vi "Calc Velocity Setpoints.vi"(7 "Autos":T6, 8 "Iterations":i32, 9 "Angle":dbl, 10 "V Scale":dbl=1.0) -> (0 "tick count(ms)":u32, 1 "Finished?":bool, 2 "setpoints":cluster{"left":dbl, "right":dbl})   [LabVIEW 2023]
uses:
  bordeaux-main/Bordeaux/Types/Single Cmd Info.ctl
  <vilib>/picture/picture.llb/imagedata.ctl
  bordeaux-main/Bordeaux/Types/Trajectory Data.ctl
  bordeaux-main/Bordeaux/Types/Segment Type.ctl
  <vilib>/addons/control/pid/pid.llb/PID (DBL).vi
  <vilib>/addons/control/pid/NI_PID_pid.lvlib
panel:
  in  "IMU PID":T1={"proportional gain (Kc)"=0.06, "integral time (Ti, min)"=0.0, "derivative time (Td, min)"=0.001}
  in  "Turn Scale":dbl=1.0
  in  "Half Track Width (ft)":dbl=0.9
  in  "IMU Correction":bool=TRUE
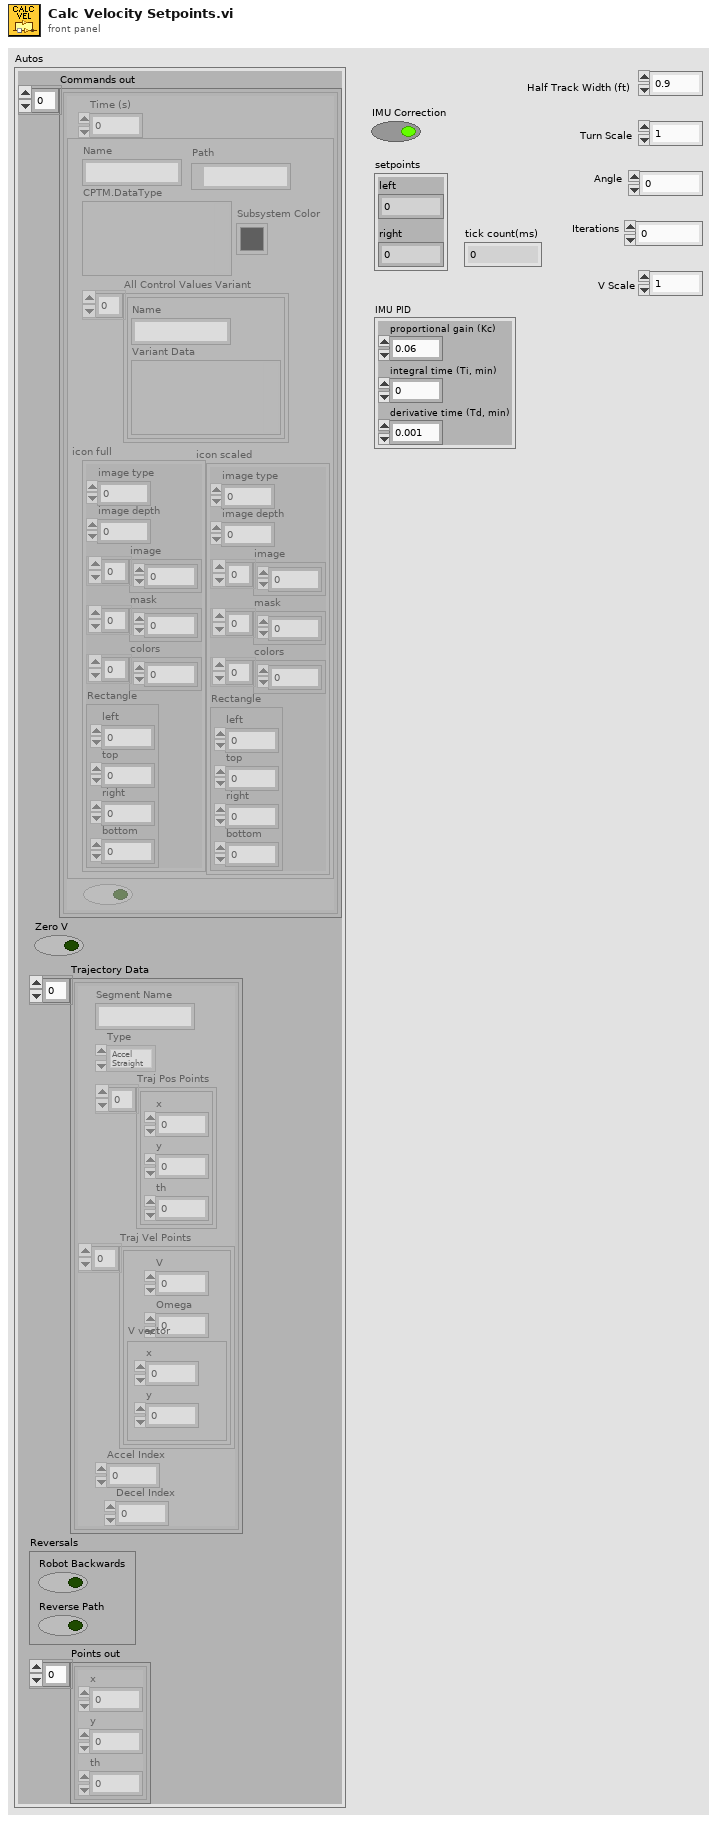
[diagram p1: front panel]
types:
  T1 = cluster{"proportional gain (Kc)":dbl, "integral time (Ti, min)":dbl, "derivative time (Td, min)":dbl}
  T2 = typedef "Single Cmd Info.ctl" = cluster{"Name":string, "CPTM.DataType":variant, "All Control Values Variant":cluster{"Name":string, "Variant Data":variant}[], "icon full":T3, "icon scaled":T3, "Path":path, "Subsystem Color":u32}
  T3 = typedef "imagedata.ctl" = cluster{"image type":i32, "image depth":i32, "image":u8[], "mask":u8[], "colors":u32[], "Rectangle":cluster{"left":i16, "top":i16, "right":i16, "bottom":i16}}
  T4 = typedef "Trajectory Data.ctl" = cluster{"Segment Name":string, "Type":T5, "Traj Pos Points":cluster{"x":dbl, "y":dbl, "th":dbl}[], "Traj Vel Points":cluster{"V":dbl, "Omega":dbl, "V vector":cluster{"y":dbl, "x":dbl}}[], "Accel Index":i32, "Decel Index":i32}[]
  T5 = typedef "Segment Type.ctl" = enum16{"Accel Straight", "Const Straight", "Blend", "Circle", "Bezier"}
  T6 = cluster{"Commands out":cluster{"Time (s)":dbl, T2, bool}[], "Zero V":bool, "Trajectory Data":T4, "Reversals":cluster{"Robot Backwards":bool, "Reverse Path":bool}, "Points out":cluster{"x":dbl, "y":dbl, "th":dbl}[]}
  T7 = cluster{"Robot Backwards":bool, "Reverse Path":bool}
  T8 = cluster{"V":dbl, "Omega":dbl, "V vector":cluster{"y":dbl, "x":dbl}}[]
  T9 = cluster{"V":dbl, "Omega":dbl, "V vector":cluster{"y":dbl, "x":dbl}}
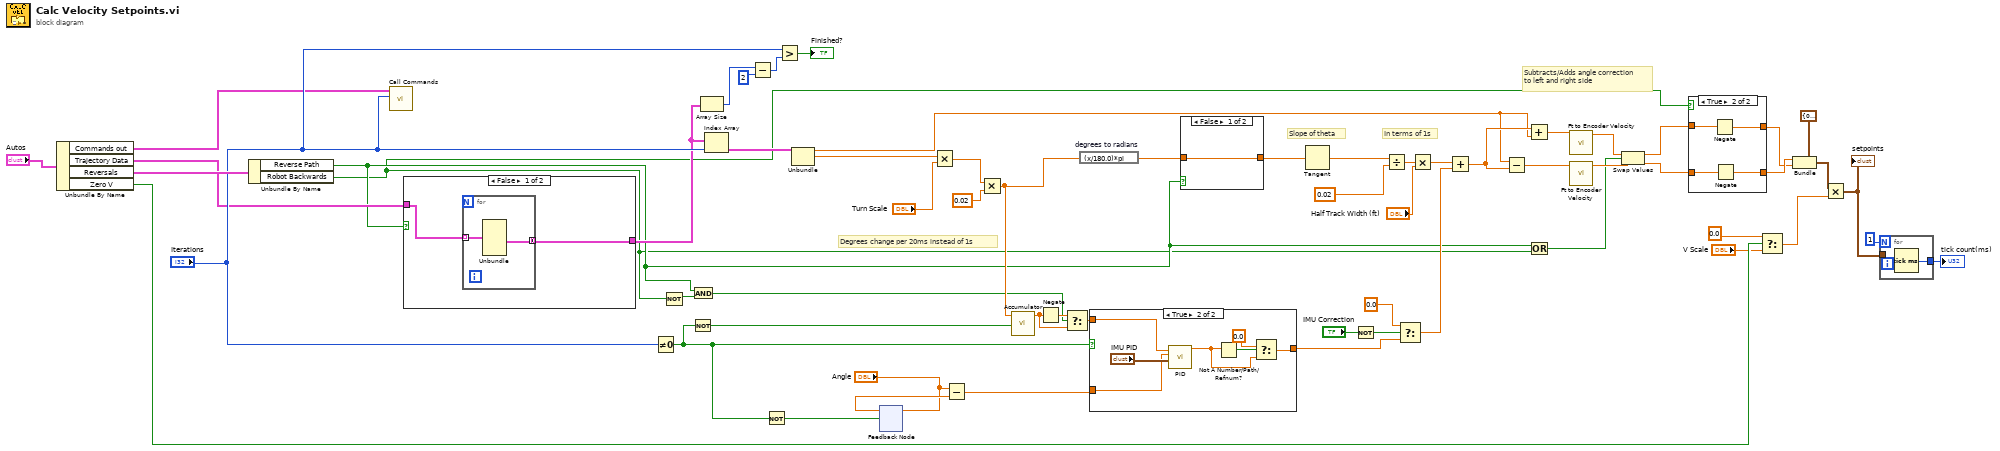
[diagram p0: block diagram]
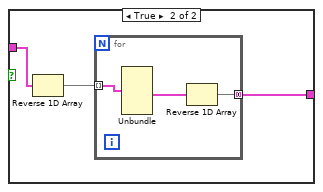
[diagram p2: hidden frame]
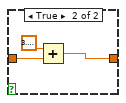
[diagram p3: hidden frame]
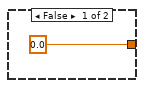
[diagram p4: hidden frame]
diagram:
  # "In terms of 1s"
  # "Slope of theta"
  # "Subtracts/Adds angle correction\nto left and right side"
  # "Degrees change per 20ms instead of 1s"
  n1 = Unbundle By Name("Autos") -> ("Commands out"=w18:cluster{"Time (s)":dbl, T2, bool}[], "Trajectory Data"=w30:T4, "Reversals"=w40:T7, "Zero V"=w17:bool)
  n2 = Unbundle By Name(w40) -> ("Reverse Path"=w3:bool, "Robot Backwards"=w2:bool)
  n3 = call "Call Commands.vi"("Iterations"="Iterations", "Commands"=w18) -> ()  [unwired: 10 in]
  n4 = case shown="False" w3 {
    tunnel: w30 -> [w63 w68]
    tunnel: [w62 w66] -> w32
    frame False {
      n5 = for {
        tunnel: w63 -> [w65] mode=indexing
        tunnel: [w64] -> w62 mode=concatenating
        n6 = Unbundle(w65) -> ("Traj Vel Points"=w64:T8)  [unwired: 5 out]
      }
    }
    frame True {
      n7 = Reverse 1D Array(array=w68) -> (reversed array=w67:T4)
      n8 = for {
        tunnel: w67 -> [w71] mode=indexing
        tunnel: [w69] -> w66 mode=concatenating
        n9 = Unbundle(w71) -> ("Traj Vel Points"=w70:T8)  [unwired: 5 out]
        n10 = Reverse 1D Array(array=w70) -> (reversed array=w69:T8)
      }
    }
  }
  n11 = Not Equal To 0?(x="Iterations") -> (x != 0?=w48:bool)
  n12 = Not(x=w2) -> (.not. x?=w8:bool)
  n13 = Not(x=w48) -> (.not. x?=w47:bool)
  n14 = And(x=w3, y=w8) -> (x .and. y?=w5:bool)
  n15 = Array Size(array=w32) -> (size(s)=w36:i32)
  n16 = Index Array(array=w32, index="Iterations") -> (element=w34:T9)
  n17 = Subtract(x=w36, y=2) -> (x-y=w50:i32)
  n18 = Not(x=w48) -> (.not. x?=w42:bool)
  n19 = Greater?(x="Iterations", y=w50) -> (0:→"Finished?":bool)
  n20 = Unbundle(w34) -> ("V"=w33:dbl, "Omega"=w9:dbl)  [unwired: 1 out]
  n21 = feedback #1() -> (w41:dbl)  [unwired: 1 in]
  n22 = feedback-in #1("Angle", w42) -> ()
  n23 = Multiply(x=w9, y="Turn Scale") -> (x*y=w24:dbl)
  n24 = Subtract(x="Angle", y=w41) -> (x-y=w22:dbl)
  n25 = Multiply(x=w24, y=0.02) -> (x*y=w21:dbl)
  n26 = call "Accumulator.vi"("Reset?"=w47, "Value"=w21) -> ("Sum"=w6:dbl)  [unwired: 9 in]
  n27 = Negate(x=w6) -> (-x=w7:dbl)
  n28 = Select(t=w7, s=w5, f=w6) -> (s? t:f=w4:dbl)
  n29 = expression code="(x/180.0)*pi" "degrees to radians"(w21) -> (w61:dbl)
  n30 = case shown="True" w48 {
    tunnel: w22 -> [_ w78]
    tunnel: w4 -> [_ w77]
    tunnel: [0.0 ("output") w73] -> w20
    frame False {
    }
    frame True {
      n31 = call-poly <vilib>:"PID.vi"("PID gains"="IMU PID", "process variable"=w78, "setpoint"=w77) -> ("output"=w75:dbl)  [unwired: 7 in, 1 out]
      n32 = Not A Number/Path/Refnum?(number/path/refnum=w75) -> (NaN/Path/Refnum?=w76:bool)
      n33 = Select(t=0.0, s=w76, f=w75) -> (s? t:f=w73:dbl)
    }
  }
  n34 = case shown="False" w3 {
    tunnel: w61 -> [w80 w83]
    tunnel: [w80 w81] -> w60
    frame False {
    }
    frame True {
      n35 = Add(x=3.141592653589793, y=w83) -> (x+y=w81:dbl)
    }
  }
  n36 = Tangent(1:w60) -> (0:w59:dbl)
  n37 = Not(x="IMU Correction") -> (.not. x?=w10:bool)
  n38 = Divide(x=w59, y=0.02) -> (x/y=w57:dbl)
  n39 = Select(t=0.0, s=w10, f=w20) -> (s? t:f=w28:dbl)
  n40 = Multiply(x=w57, y="Half Track Width (ft)") -> (x*y=w46:dbl)
  n41 = Add(x=w46, y=w28) -> (x+y=w45:dbl)
  n42 = Subtract(x=w33, y=w45) -> (x-y=w26:dbl)
  n43 = Add(x=w45, y=w33) -> (x+y=w25:dbl)
  n44 = Or(x=w3, y=w2) -> (x .or. y?=w1:bool)
  n45 = call "Ft to Encoder Velocity.vi"("ft/s"=w25) -> ("v"=w56:dbl)  [unwired: 10 in]
  n46 = call "Ft to Encoder Velocity.vi"("ft/s"=w26) -> ("v"=w55:dbl)  [unwired: 10 in]
  n47 = Swap Values(12:w56, 13:w1, 14:w55) -> (1:w54:dbl, 3:w53:dbl)
  n48 = case shown="True" w2 {
    tunnel: w54 -> [w85 w89]
    tunnel: w53 -> [w84 w88]
    tunnel: [w85 w87] -> w12
    tunnel: [w84 w86] -> w13
    frame False {
    }
    frame True {
      n49 = Negate(x=w89) -> (-x=w87:dbl)
      n50 = Negate(x=w88) -> (-x=w86:dbl)
    }
  }
  n51 = Select(t=0.0, s=w17, f="V Scale") -> (s? t:f=w14:dbl)
  n52 = Bundle(cluster=cluster{"left":dbl, "right":dbl} {"left"=0.0, "right"=0.0} ("setpoints"), "left"=w13, "right"=w12) -> (w49:cluster{"left":dbl, "right":dbl})
  n53 = Multiply(x=w49, y=w14) -> (x*y=w38:cluster{"left":dbl, "right":dbl})
  "setpoints" <- w38
  n54 = for {
    N: 1 -> [_]
    tunnel: w38 -> [_]
    tunnel: [w90] -> w39
    n55 = Tick Count (ms)() -> (millisecond timer value=w90:u32)
  }
  "tick count(ms)" <- w39
